vi "test_moteurs_roues.vi"   [LabVIEW 2017]
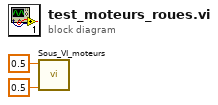
[diagram p0: block diagram]
diagram:
  n1 = call "Sous_VI_moteurs.vi"("Moteur Droit"=0.5, "Moteur Gauche"=0.5) -> ()  [unwired: 10 in]
